vi "Reference Template.vi"(8 "error in":errorcluster, 11 "ToastBuilder in":refnum<class "ToastBuilder.lvclass">) -> (0 "error out":errorcluster, 3 "ToastBuilder out":refnum<class "ToastBuilder.lvclass">)   [LabVIEW 2026, in "ToastNotification.lvlib" / "ToastBuilder.lvclass"]
doc: "Private authoring template containing native class property nodes for Builder Reference. On no incoming error, read and write the same handle; on error, pass the class and error through. Does not initialize, display or close a toast. This template is not an application entry point."
uses:
  ToastBuilder.lvclass
  ToastBuilder.lvclass/ToastBuilder.ctl
  Read Builder Reference.vi
  Write Builder Reference.vi
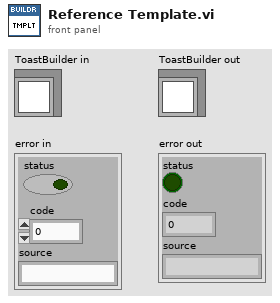
[diagram p1: front panel]
types:
  T1 = typedef "ToastNotification.lvlib/ToastBuilder.lvclass/Builder Reference.ctl" = refnum<k24>
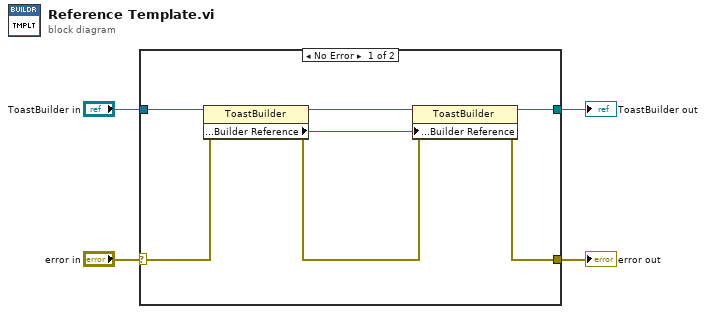
[diagram p0: block diagram]
diagram:
  n1 = case shown="No Error" "error in" {
    selector: "error in" -> [w9 w12]
    tunnel: "ToastBuilder in" -> [w11 w13]
    tunnel: [w8 w13] -> w2
    tunnel: [w6 w12] -> w1
    frame No Error {
      n2 = property class="ToastBuilder"(reference=w11, error in=w9) -> (reference out=w10:refnum<class "ToastBuilder.lvclass">, error out=w7:errorcluster, "Public:Properties:Builder Reference"=w5:T1)
      n3 = property class="ToastBuilder"(reference=w10, error in=w7, "Public:Properties:Builder Reference"=w5) -> (reference out=w8:refnum<class "ToastBuilder.lvclass">, error out=w6:errorcluster)
    }
    frame Error {
    }
  }
  "ToastBuilder out" <- w2
  "error out" <- w1
